vi "macro_LinearSystem_Sim_Execute.vi"() -> ()   [LabVIEW 2019, in "Trajectory_Library.lvlib"]
uses:
  Trajectory_Library.lvlib
  TypeDef/LINEAR_SYSTEM.ctl
  <vilib>/Analysis/Matrix/Datatypes/RealMatrix.ctl
  BatterySim_CalculateLoadedBatteryVoltage.vi
  <vilib>/Analysis/Matrix/NI_Matrix.lvlib
panel:
  in  "Demand Array (CO)":dbl[](array[numeric])
  in  "Linear System":T1
  in  "Current":dbl
  # "<States,States>"
  # "<States,Inputs>"
  # "<Outputs,States>"
  # "<Outputs,Inputs>"
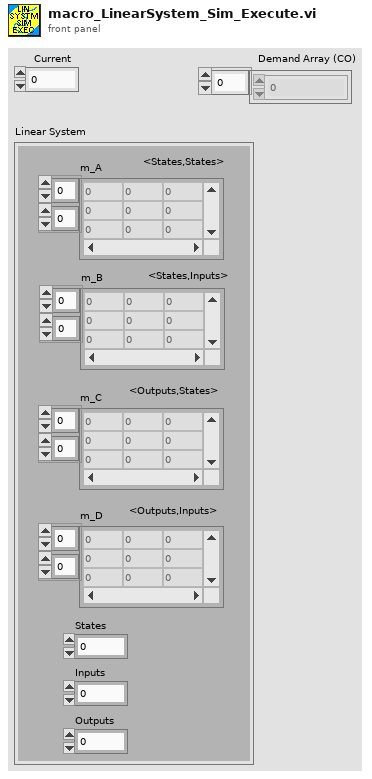
[diagram p1: front panel]
types:
  T1 = typedef "Trajectory_Library.lvlib/LINEAR_SYSTEM.ctl" = cluster{"m_A":T2, "m_B":T2, "m_C":T2, "m_D":T2, "States":i32, "Inputs":i32, "Outputs":i32}
  T2 = typedef "NI_Matrix.lvlib/RealMatrix.ctl" = dbl[][]
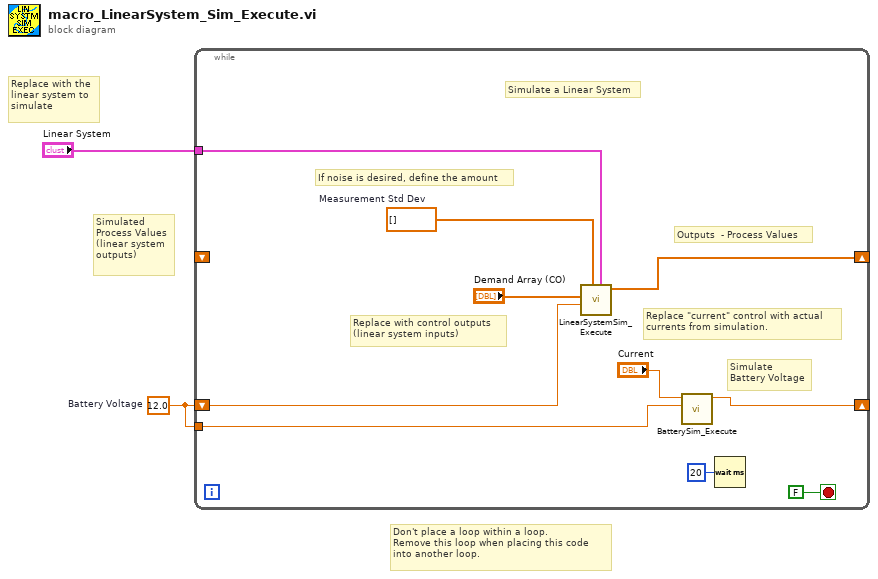
[diagram p0: block diagram]
diagram:
  w1 = 12.0  # Battery Voltage
  # "Replace with the\nlinear system to \nsimulate"
  # "Don't place a loop within a loop. \nRemove this loop when placing this code\ninto another loop."
  # "Simulated\nProcess Values\n(linear system\noutputs)"
  n1 = while {
    shift-right: [w10] -> _
    shift-left: w1 -> [w8]
    shift-right: [w9] -> _
    shift-left: _ -> [_]
    tunnel: "Linear System" -> [w6]
    tunnel: w1 -> [w3]
    stop <- FALSE stop-if-true
    w5 = dbl[] []  # Measurement Std Dev
    # "If noise is desired, define the amount"
    # "Replace \"current\" control with actual\ncurrents from simulation."
    # "Outputs  - Process Values"
    # "Replace with control outputs\n(linear system inputs)"
    # "Simulate\nBattery Voltage"
    # "Simulate a Linear System"
    n2 = call "LinearSystemSim_Execute.vi"("Linear System"=w6, "Measurement Std Dev"=w5, "Battery Voltage"=w8, "Demand Array (CO)"="Demand Array (CO)") -> ("Outputs"=w9:dbl[])  [unwired: 5 in, 2 out]
    n3 = call "BatterySim_Execute.vi"("Nominal Battery Voltage"=w3, "Current"="Current") -> ("Voltage"=w10:dbl)  [unwired: 9 in]
    n4 = Wait (ms)(milliseconds to wait=u32 20) -> ()  [unwired: 1 out]
  }
